vi "SA set Marker NextPeak.vi"(8 "error in (no error)":errorcluster caption="에러 입력(에러 없음)", 10 "Marker Index":i32, 11 "Instrument Manager 입력":refnum<class "Instrument Manager.lvclass">) -> (0 "error out":errorcluster caption="에러 출력", 3 "Instrument Manager 출력":refnum<class "Instrument Manager.lvclass">)   [LabVIEW 2023, in "Instrument Manager.lvclass"]
uses:
  Instrument Manager.lvclass
  Module/Spectrum Analyzer/Class/FSV-40N/FSV-40N.lvclass
  Instrument Manager.lvclass/Instrument Manager.ctl
  Module/Spectrum Analyzer/Class/FSV-40N/FSV-40N.lvclass/FSV-40N.ctl
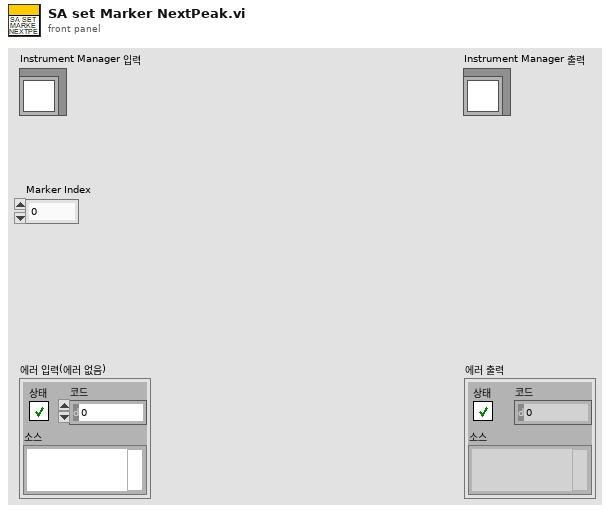
[diagram p1: front panel]
types:
  T1 = cluster{"Anritsu Call Box":refnum<class "Anritsu Call Box.lvclass">, "Spectrum Analyzer":refnum<class "Interface_Spectrum.lvclass">, "RF Switch Box":refnum<class "RF Filter Box.lvclass">, "Turn Table":refnum<class "Interface - Turn Table.lvclass">, "Mast":refnum<class "Interface - Mast.lvclass">, "3D Controller":refnum<class "Interface_3D Controller.lvclass">}
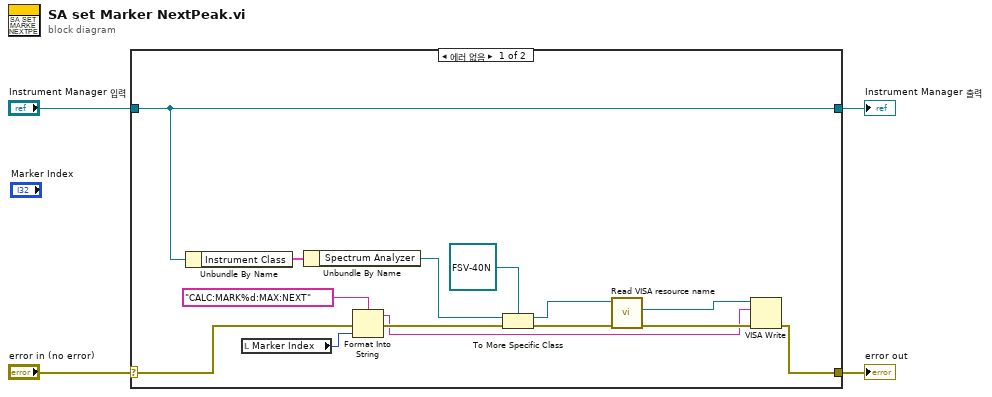
[diagram p0: block diagram]
diagram:
  n1 = case shown="에러 없음" "error in (no error)" {
    selector: "error in (no error)" -> [w9 w20]
    tunnel: [w8 w20] -> w3
    tunnel: [w18 w19] -> w1
    tunnel: "Instrument Manager 입력" -> [w18 w19]
    frame No Error {
      n2 = Unbundle By Name(w18) -> ("Instrument Class"=w17:T1)
      n3 = local read "Marker Index"() -> (w7:i32)
      n4 = Unbundle By Name(w17) -> ("Spectrum Analyzer"=w10:refnum<class "Interface_Spectrum.lvclass">)
      n5 = Format Into String(format string="CALC:MARK%d:MAX:NEXT" ("initial string"), error in=w9, w7) -> (resulting string=w5:string, error out=w16:errorcluster)  [unwired: 1 in]
      n6 = To More Specific Class(target class=refnum<class "FSV-40N.lvclass"> refnum ("Spectrum Analyzer.lvlib:FSV-40N.lvclass"), reference=w10, error in=w16) -> (specific class reference=w13:refnum<class "FSV-40N.lvclass">, error out=w14:errorcluster)
      n7 = call "Read VISA resource name.vi"("error in (no error)"=w14, "FSV-40N in"=w13) -> ("error out"=w12:errorcluster, "VISA resource name"=w11:refnum<visa-resource-name>)  [unwired: 7 in, 1 out]
      n8 = VISA Write(VISA resource name=w11, write buffer=w5, error in (no error)=w12) -> (error out=w8:errorcluster)  [unwired: 2 out]
    }
    frame Error {
    }
  }
  "error out" <- w3
  "Instrument Manager 출력" <- w1
